vi "decoder_lfsr.vi"() -> ()   [LabVIEW 2025]
panel:
  out "Message":u32 format="%b"
  in  "Message with CRC":u32 format="%b"
  out "CRC":u32 format="%b"
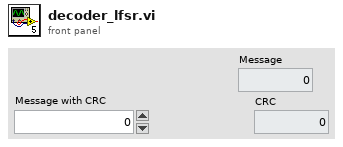
[diagram p1: front panel]
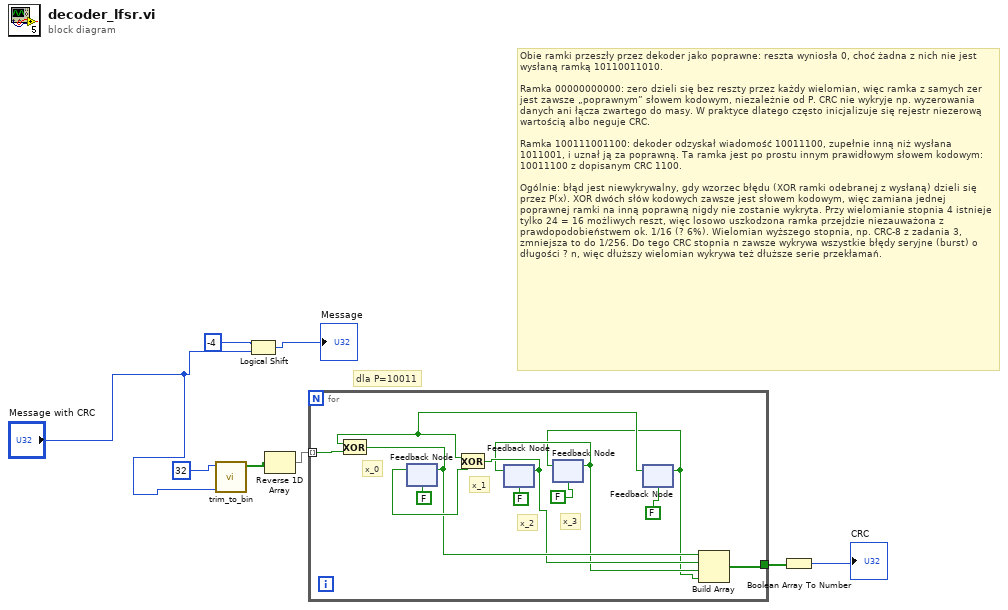
[diagram p0: block diagram]
diagram:
  # "Obie ramki przeszły przez dekoder jako poprawne: reszta wyniosła 0, choć żadna z nich nie jest wysłaną ramką 10110011010.\n\nRamka 00000000000: zero dzieli się bez reszty przez każdy wielomian, więc ramka z samych zer jest zawsze „poprawnym” słowem kodowym, niezależnie od P. CRC nie wykryje np. wyzerowania danych ani łącza zwartego do masy. W praktyce dlatego często inicjalizuje się rejestr niezerową wartością albo neguje CRC.\n\nRamka 100111001100: dekoder odzyskał wiadomość 10011100, zupełnie inną niż wysłana 1011001, i uznał ją za poprawną. Ta ramka jest po prostu innym prawidłowym słowem kodowym: 10011100 z dopisanym CRC 1100.\n\nOgólnie: błąd jest niewykrywalny, gdy wzorzec błędu (XOR ramki odebranej z wysłaną) dzieli się przez P(x). XOR dwóch słów kodowych zawsze jest słowem kodowym, więc zamiana jednej poprawnej ramki na inną poprawną nigdy nie zostanie wykryta. Przy wielomianie stopnia 4 istnieje tylko 24 = 16 możliwych reszt, więc losowo uszkodzona ramka przejdzie niezauważona z prawdopodobieństwem ok. 1/16 (? 6%). Wielomian wyższego stopnia, np. CRC-8 z zadania 3, zmniejsza to do 1/256. Do tego CRC stopnia n zawsze wykrywa wszystkie błędy seryjne (burst) o długości ? n, więc dłuższy wielomian wykrywa też dłuższe serie przekłamań."
  # "dla P=10011"
  n1 = call "trim_to_bin.vi"("number"="Message with CRC", "constant"=u32 32) -> ("new array"=w7:bool[])  [unwired: 8 in, 1 out]
  n2 = Logical Shift(y=i16 -4, x="Message with CRC") -> (x << y=→"Message":u32)
  n3 = Reverse 1D Array(array=w7) -> (reversed array=w6:bool[])
  n4 = for {
    tunnel: w6 -> [w20] mode=indexing
    tunnel: [w13] -> w5
    # "x_3"
    # "x_2"
    # "x_1"
    # "x_0"
    n5 = feedback #1(FALSE) -> (w14:bool)
    n6 = feedback #2(FALSE) -> (w10:bool)
    n7 = feedback #3(FALSE) -> (w9:bool)
    n8 = feedback-in #3(w10) -> ()
    n9 = feedback #4(FALSE) -> (w15:bool)
    n10 = Exclusive Or(1:w20, 2:w15) -> (0:w12:bool)
    n11 = feedback-in #1(w12) -> ()
    n12 = Exclusive Or(1:w14, 2:w15) -> (0:w11:bool)
    n13 = feedback-in #2(w11) -> ()
    n14 = feedback-in #4(w9) -> ()
    n15 = Build Array(w12, w11, w10, w9) -> (w13:bool[])
  }
  n16 = Boolean Array To Number(Boolean array=w5) -> (number=→"CRC":u32)
